vi "PLC Sim Launcher.vi"() -> ()   [LabVIEW 2025]
uses:
  PLC Sim Controller/PLC Sim Controller/PLC Sim Controller Actor.lvclass
  C:/Program Files/National Instruments/LabVIEW 2025/vi.lib/ActorFramework/Actor/Actor.lvclass
  f3c1f790-3e5d-4544-8d8b-87c596bc95fa.vi
  <vilib>/ActorFramework/Actor/Actor.lvclass
panel:
  out "Waiting Lights":T1
  # "PLC Simulated Server"
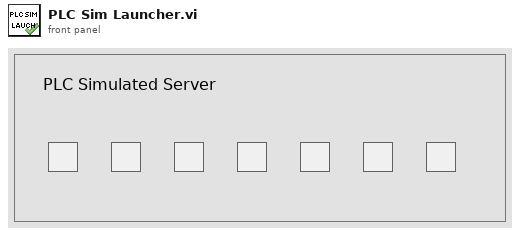
[diagram p1: front panel]
types:
  T1 = cluster{"Wait 1":bool, "Wait 2":bool, "Wait 3":bool, "Wait 4":bool, "Wait 5":bool, "Wait 6":bool, "Wait 7":bool}
  T2 = cluster{"[0]":bool, "[1]":bool, "[2]":bool, "[3]":bool, "[4]":bool, "[5]":bool, "[6]":bool}
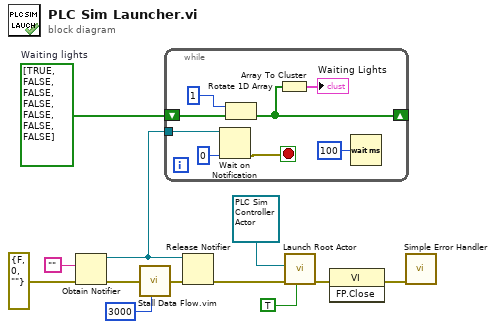
[diagram p0: block diagram]
diagram:
  w9 = bool[] [TRUE, FALSE, FALSE, FALSE, FALSE, FALSE, FALSE]  # Waiting lights
  n1 = Obtain Notifier(notification data type="", error in (no error)=errorcluster {"status"=FALSE, "code"=0, "source"=""}) -> (notifier out=w6:refnum<notifier>, error out=w5:errorcluster)  [unwired: 2 in, 1 out]
  n2 = call "Stall Data Flow.vim"("value in"=w5, "milliseconds to wait"=u32 3000) -> ("value out"=w10:errorcluster)  [unwired: 1 out]
  n3 = while {
    shift-right: [w14] -> _
    shift-left: w9 -> [w16]
    tunnel: w6 -> [w18]
    stop <- w20 stop-if-true
    n4 = Wait on Notification(notifier=w18, timeout in ms (-1)=0) -> (error out=w20:errorcluster)  [unwired: 2 in, 3 out]
    n5 = Rotate 1D Array(1:w16, 2:1 ("n")) -> (0:w14:bool[])
    n6 = Array To Cluster(array=w14) -> (cluster=→"Waiting Lights":T2)
    n7 = Wait (ms)(milliseconds to wait=u32 100) -> ()  [unwired: 1 out]
  }
  n8 = Release Notifier(notifier=w6, error in (no error)=w10) -> (error out=w4:errorcluster)  [unwired: 1 in, 2 out]
  n9 = call <vilib>:"Launch Root Actor.vi"("Open Actor Core front panel? (F)"=TRUE, "error in (no error)"=w4, "Actor"=refnum<class "PLC Sim Controller Actor.lvclass"> refnum ("PLC Sim Controller Actor.lvlib:PLC Sim Controller Actor.lvclass")) -> ("error out"=w3:errorcluster)  [unwired: 7 in, 1 out]
  n10 = invoke class="VI" method="FP.Close"(error in=w3) -> (error out=w1:errorcluster)  [unwired: 2 in, 2 out]
  n11 = call <vilib>:"Simple Error Handler.vi"("error in (no error)"=w1) -> ()  [unwired: 4 in, 5 out]
